vi "EditCellValue.vi"(0 "VI Reference In":refnum<vi>, 2 "delimiter (>>)":string=">>", 5 "Control Path":string, 7 "Row Index":i32, 9 "Value":string, 11 "Error In":errorcluster, 14 "Column Index":i32) -> (4 "VI Reference Out":refnum<vi>, 15 "Error Out":errorcluster)   [LabVIEW 2016, in "Drona.lvlib" / "ControlValue.lvlib" / "StimulusTable.lvlib"]
doc: "Sets value(signaling) for the table control whose cell index is specified. \n\nThe input control name is given as a string , incase of path, use delimiters inbetween the path.\n\nThis node generates error if used for an empty table."
uses:
  StimulusTable.lvlib
  <vilib>/Utility/error.llb/Error Cluster From Error Code.vi
  <vilib>/ErrorRing/Error Ring.xnode
  Drona.lvlib
  Get/GetControlRef/GetControlRef.lvlib
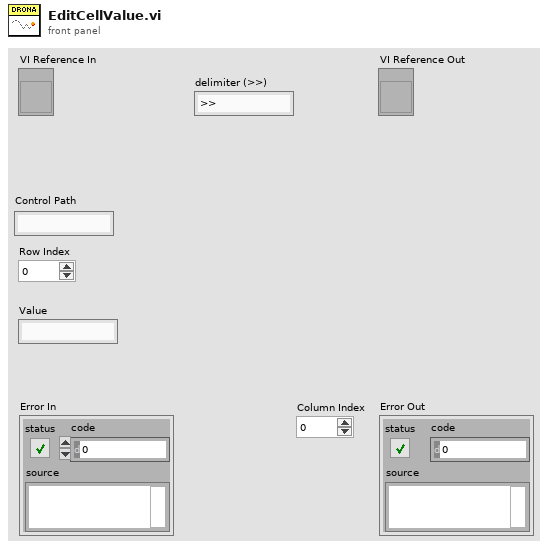
[diagram p1: front panel]
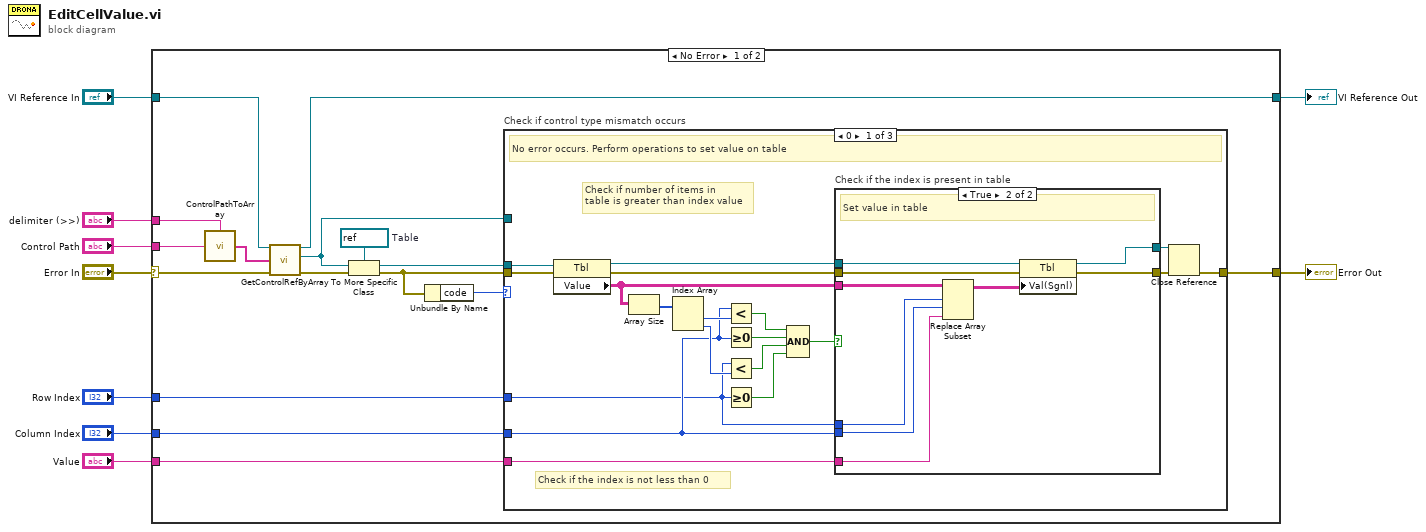
[diagram p0: block diagram]
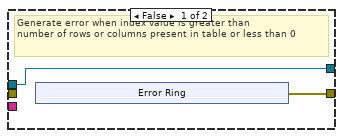
[diagram p2: hidden frame]
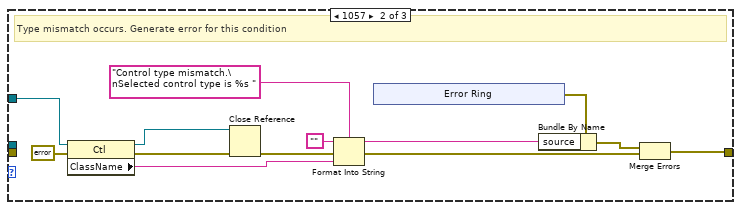
[diagram p3: hidden frame]
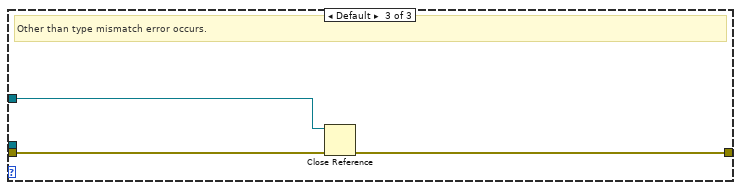
[diagram p4: hidden frame]
diagram:
  n1 = case shown="No Error" "Error In" {
    selector: "Error In" -> [w14 w83]
    tunnel: [w22 w83] -> w8
    tunnel: "VI Reference In" -> [w18 w82]
    tunnel: "Control Path" -> [w24 _]
    tunnel: "Column Index" -> [w20 _]
    tunnel: [w17 w82] -> w4
    tunnel: "delimiter (>>)" -> [w23 _]
    tunnel: "Value" -> [w11 _]
    tunnel: "Row Index" -> [w10 _]
    frame No Error {
      w25 = refnum<vi> refnum  # Table
      n2 = call "ControlPathToArray.vi"("Control Name"=w24, "delimiter (>>)"=w23) -> ("Control Path"=w19:string[])
      n3 = call "GetControlRefByArray.vi"("VI Reference In"=w18, "Control Path"=w19, "error In"=w14) -> ("VI Reference Out"=w17:refnum<vi>, "Ctl Refnum"=w15:refnum<vi>, "error out"=w16:errorcluster)  [unwired: 10 in]
      n4 = To More Specific Class(target class=w25, reference=w15, error in=w16) -> (specific class reference=w21:refnum<vi>, error out=w13:errorcluster)
      n5 = Unbundle By Name(w13) -> ("code"=w12:i32)
      n6 = case "Check if control type mismatch occurs" shown="0" w12 {
        tunnel: [w44 w63 w80] -> w22
        tunnel: w21 -> [w39 _ _]
        tunnel: w20 -> [w28 _ _]
        tunnel: w15 -> [_ w73 w79]
        tunnel: w13 -> [w43 _ w81]
        tunnel: w11 -> [w37 _ _]
        tunnel: w10 -> [w27 _ _]
        frame 0 {
          # "Check if number of items in \ntable is greater than index value"
          # "Check if the index is not less than 0"
          # "No error occurs. Perform operations to set value on table"
          n7 = property class="Tbl"(reference=w39, error in=w43) -> (reference out=w38:refnum<vi>, error out=w40:errorcluster, "Value"=w29:string[][])
          n8 = Array Size(array=w29) -> (size(s)=w32:i32[])
          n9 = Index Array(array=w32) -> (element #1=w31:i32, element #2=w30:i32)  [unwired: 2 in]
          n10 = Less?(x=w28, y=w31) -> (x < y?=w36:bool)
          n11 = Greater Or Equal To 0?(x=w28) -> (x >= 0?=w35:bool)
          n12 = Less?(x=w27, y=w30) -> (x < y?=w34:bool)
          n13 = Greater Or Equal To 0?(x=w27) -> (x >= 0?=w33:bool)
          n14 = Compound Arithmetic op=AND(w36, w35, w34, w33) -> (w26:bool)
          n15 = case "Check if the index is present in table" shown="True" w26 {
            tunnel: [w45 w59] -> w42
            tunnel: [w46 w54] -> w41
            tunnel: w40 -> [_ w60]
            tunnel: w38 -> [w46 w58]
            tunnel: w28 -> [_ w53]
            tunnel: w29 -> [_ w57]
            tunnel: w37 -> [_ w55]
            tunnel: w27 -> [_ w52]
            frame False {
              # "Generate error when index value is greater than \nnumber of rows or columns present in table or less than 0"
              n16 = xnode "Error Ring"() -> ("error out"=w45:errorcluster)
            }
            frame True {
              # "Set value in table"
              n17 = Replace Array Subset(array=w57, new element=w55, index (row)=w52, index (col)=w53) -> (w56:string[][])
              n18 = property class="Tbl"(reference=w58, error in=w60, "Val(Sgnl)"=w56) -> (reference out=w54:refnum<vi>, error out=w59:errorcluster)
            }
          }
          n19 = Close Reference(reference=w41, error in (no error)=w42) -> (error out=w44:errorcluster)
        }
        frame 1057 {
          # "Type mismatch occurs. Generate error for this condition"
          n20 = property class="Ctl"(reference=w73, error in=errorcluster {"status"=FALSE, "code"=0, "source"=""} ("error out")) -> (reference out=w61:refnum<vi>, error out=w72:errorcluster, "ClassName"=w69:string)
          n21 = Close Reference(reference=w61, error in (no error)=w72) -> (error out=w62:errorcluster)
          n22 = Format Into String(format string="Control type mismatch.\nSelected control type is %s ", initial string="", error in=w62, w69) -> (resulting string=w66:string, error out=w64:errorcluster)
          n23 = xnode "Error Ring"() -> ("error out"=w67:errorcluster)
          n24 = Bundle By Name(cluster=w67, "source"=w66) -> (w65:errorcluster)
          n25 = Merge Errors(w65, w64) -> (w63:errorcluster)
        }
        frame Default {
          # "Other than type mismatch error occurs."
          n26 = Close Reference(reference=w79, error in (no error)=w81) -> (error out=w80:errorcluster)
        }
      }
    }
    frame Error {
    }
  }
  "Error Out" <- w8
  "VI Reference Out" <- w4
